vi "BPM_Detect.vi"(0 "RMS Buffer":dbl[](array[numeric]), 4 "Sample Interval(sec)":dbl) -> (8 "BPM":dbl)   [LabVIEW 2026]
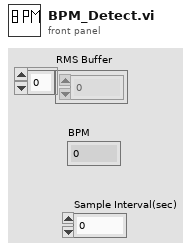
[diagram p1: front panel]
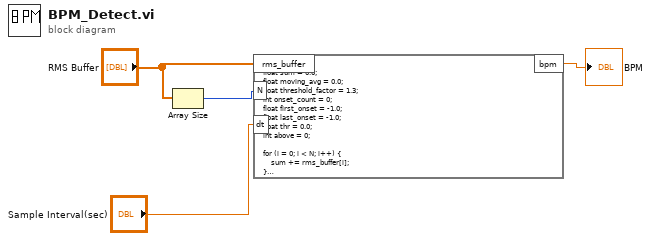
[diagram p0: block diagram]
diagram:
  n1 = Array Size(array="RMS Buffer") -> (size(s)=w1:i32)
  n2 = formula code="int i;\nfloat sum = 0.0;\nfloat moving_avg = 0.0;\nfloat threshold_factor = 1.3;\nint onset_count = 0;\nfloat first_onset = -1.0;\nfloat last_onset = -1.0;\nfloat thr = 0.0;\nint above = 0;\n\nfor (i = 0; i < N; i++) {\n    sum += rms_buffer[i];\n}\nmoving_avg = sum / N;\nthr = threshold_factor * moving_avg;\n\nfor (i = 0; i < N; i++) {\n    if (rms_buffer[i] > thr && above == 0) {\n        above = 1;\n        onset_count = onset_count + 1;\n        if (first_onset < 0.0) { first_onset = i * dt; }\n        last_onset = i * dt;\n    }\n    if (rms_buffer[i] <= thr) { above = 0; }\n}\n\nif (onset_count >= 2 && last_onset > first_onset) {\n    bpm = 60.0 * (onset_count - 1) / (last_onset - first_onset);\n} else {\n    bpm = 0.0;\n}"("rms_buffer"="RMS Buffer", "N"=w1, "dt"="Sample Interval(sec)") -> ("bpm"=→"BPM":dbl)
